vi "PWM_Write_Ex.vi"() -> ()   [LabVIEW 2026]
panel:
  in  "Duty Cycle":u8(slide) scale=0.0..255.0
  in  "Canal":u8
  in  "Stop Button":bool
  out "error out":errorcluster
  out "respuesta":string
  in  "VISA resource name":refnum<visa-resource-name>
  # "Ejemplo: PWM Write"
  # "Descripcion: Genera una señal PWM en un pin del microcontrolador controlando el ciclo de trabajo."
  # "Configuracion"
  # "Indicadores"
  # "Control"
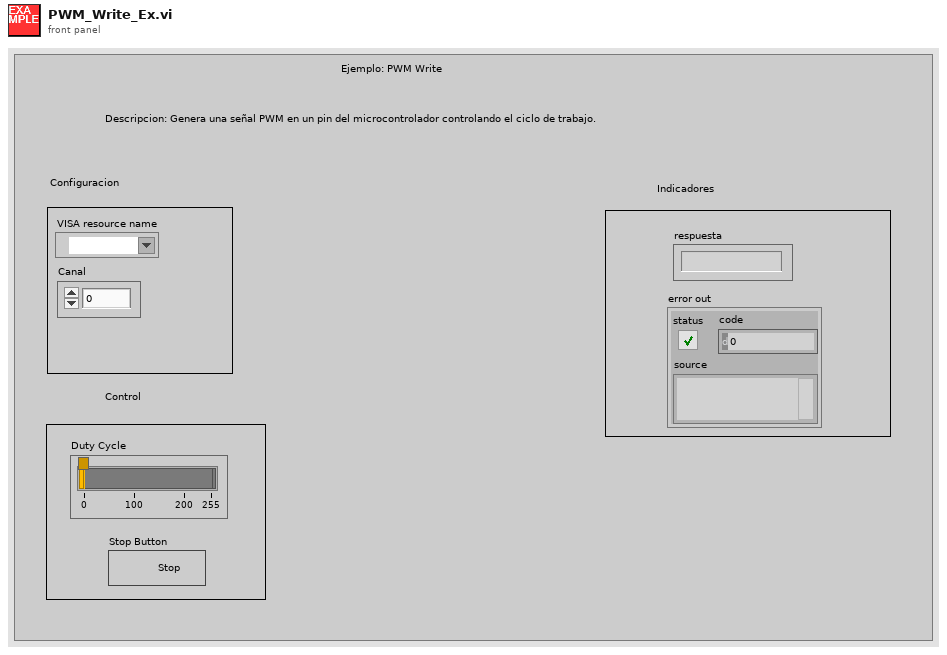
[diagram p1: front panel]
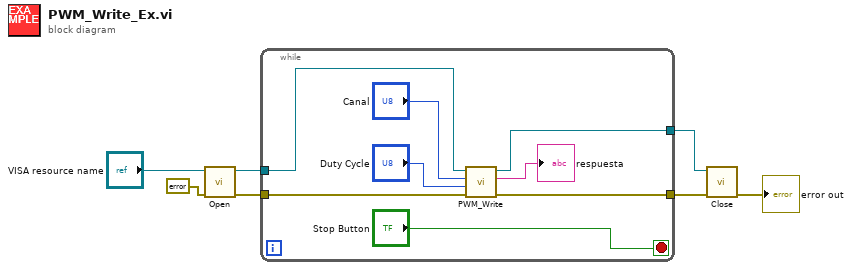
[diagram p0: block diagram]
diagram:
  n1 = call "Open.vi"("error in (no error)"=errorcluster {"status"=FALSE, "code"=0, "source"=""}, "VISA resource name"="VISA resource name") -> ("error out"=w5:errorcluster, "VISA resource name out"=w4:refnum<visa-resource-name>)  [unwired: 8 in]
  n2 = while {
    tunnel: w4 -> [w14]
    tunnel: [w13] -> w3
    tunnel: w5 -> [w15]
    tunnel: [w12] -> w2
    stop <- "Stop Button" stop-if-true
    n3 = call "PWM_Write.vi"("error in (no error)"=w15, "Duty Cycle"="Duty Cycle", "Canal"="Canal", "VISA resource name"=w14) -> ("error out"=w12:errorcluster, "respuesta"=→"respuesta":string, "VISA resource name out"=w13:refnum<visa-resource-name>)  [unwired: 5 in]
  }
  n4 = call "Close.vi"("error in (no error)"=w2, "VISA resource name"=w3) -> ("error out"=→"error out":errorcluster)  [unwired: 9 in]
